vi "LoadCFG.vi"(8 "error in (no error)":errorcluster, 11 "object in":refnum<class "DIO-Configuration.lvclass">) -> (0 "error out":errorcluster, 2 "Success?":bool, 3 "object out":refnum<class "DIO-Configuration.lvclass">)   [LabVIEW 2021, in "DAQmx.lvlib" / "DIO-Configuration.lvclass"]
doc: "Loads Configuration"
uses:
  DIO-Configuration.lvclass
  C:/Users/averna/Documents/LV Gym DEMO/Factory Pattern/Device Channels/Dependencies/Channel.lvlibp/Channel/Configuration_class/Configuration.lvclass
  DIO-Configuration.lvclass/DIO-Configuration.ctl
  Dependencies/Channel.lvlibp/Channel/Configuration_class/properties/ReadConfigurationFile.vi
  <vilib>/Utility/config.llb/Read Key (String).vi
  Dependencies/DIO-Channel.lvlibp/DIO-Configuration_class/DIO-Configuration.lvclass
  <vilib>/Utility/config.llb/NI_LVConfig.lvlib
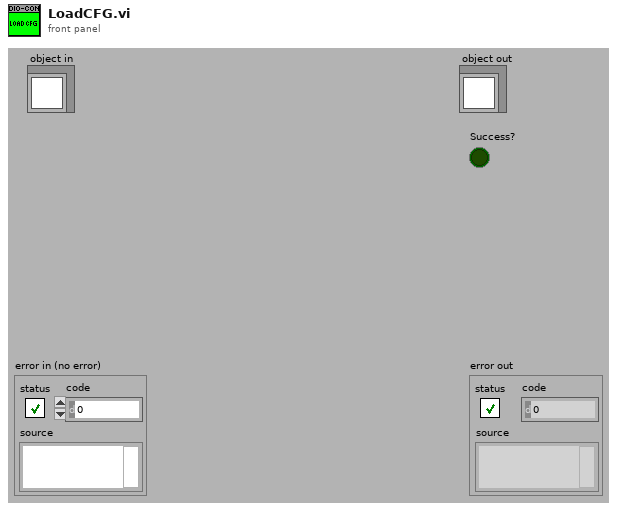
[diagram p1: front panel]
types:
  T1 = typedef "NI_LVConfig.lvlib/Config Data RefNum.ctl" = refnum<k1>
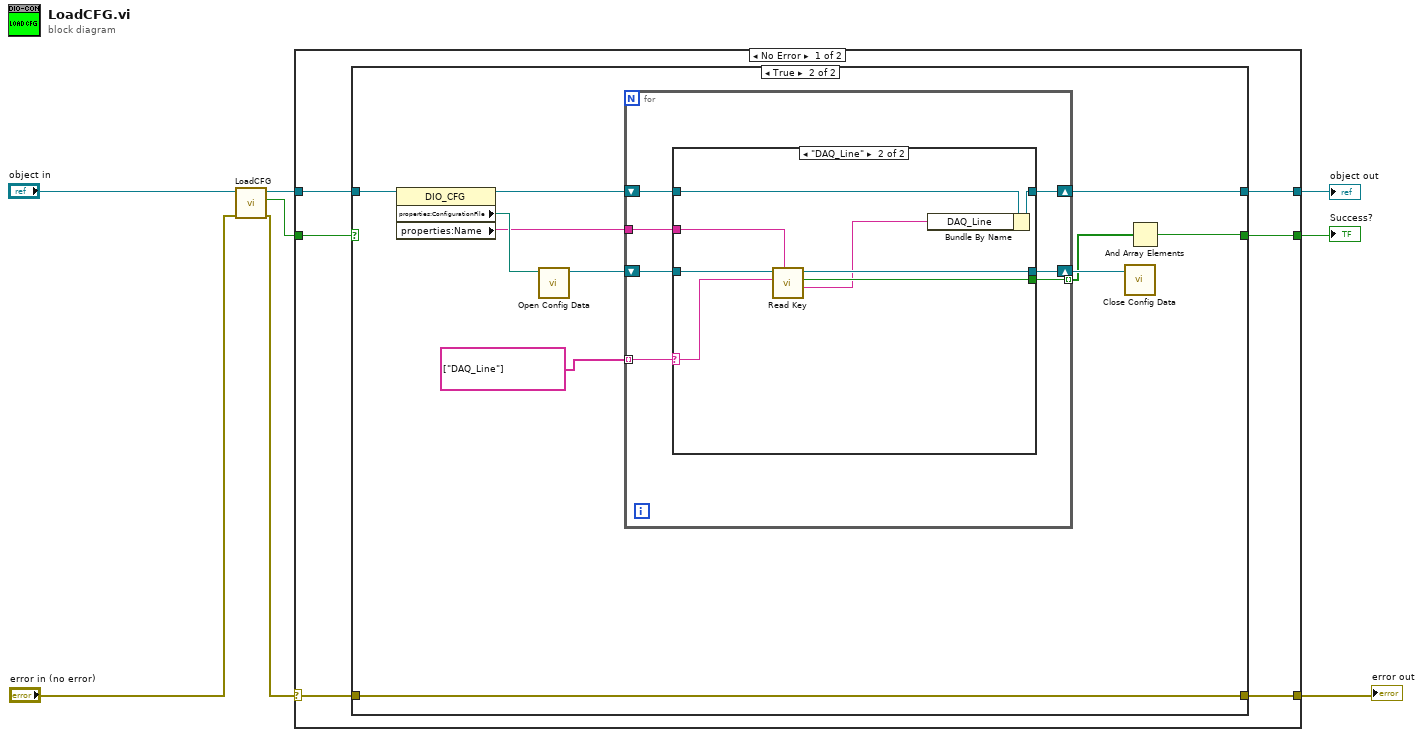
[diagram p0: block diagram]
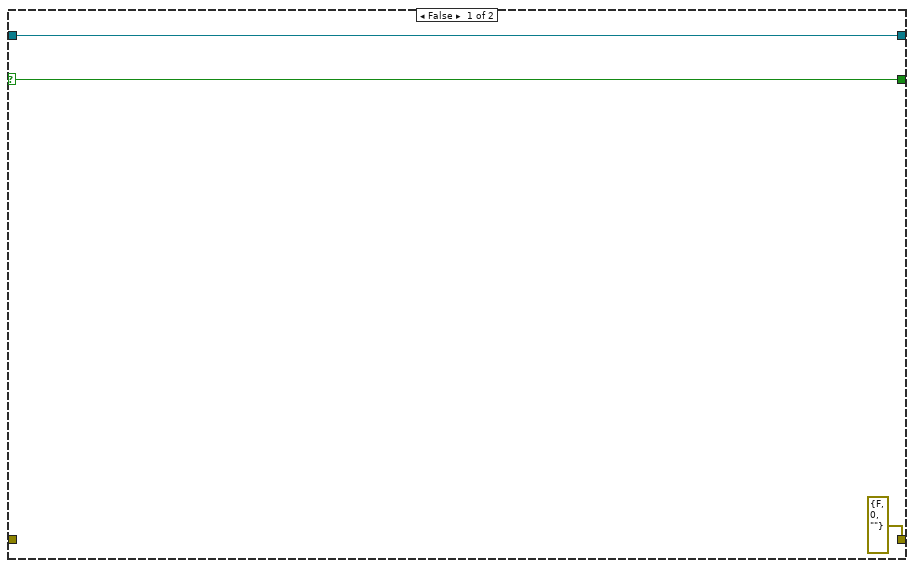
[diagram p2: hidden frame]
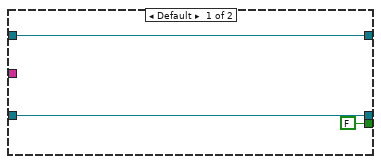
[diagram p3: hidden frame]
diagram:
  n1 = call-parent "LoadCFG.vi"("error in (no error)"="error in (no error)", "object in"="object in") -> ("error out"=w4:errorcluster, "Success?"=w5:bool, "object out"=w6:refnum<class "DIO-Configuration.lvclass">)  [unwired: 7 in]
  n2 = case shown="No Error" w4 {
    selector: w4 -> [w11 w49]
    tunnel: [w12 w49] -> w3
    tunnel: w6 -> [w13 w48]
    tunnel: [w9 w47] -> w1
    tunnel: w5 -> [w10 w47]
    tunnel: [w14 w48] -> w2
    frame No Error {
      n3 = case shown="True" w10 {
        selector: w10 -> [w16 _]
        tunnel: [w17 w24] -> w14
        tunnel: w13 -> [w17 w28]
        tunnel: [errorcluster {"status"=FALSE, "code"=0, "source"=""} ("error IO") w27] -> w12
        tunnel: w11 -> [_ w27]
        tunnel: [w16 w18] -> w9
        frame False {
        }
        frame True {
          n4 = property class="DIO_CFG"(reference=w28) -> (reference out=w23:refnum<class "DIO-Configuration.lvclass">, "properties:ConfigurationFile"=w26:path, "properties:Name"=w20:string)  [unwired: 1 in, 1 out]
          n5 = call <vilib>:"Open Config Data.vi"("configuration file path"=w26) -> ("refnum"=w25:T1)  [unwired: 8 in, 2 out]
          n6 = for {
            shift-right: [w31] -> w24
            shift-left: w23 -> [w30]
            shift-right: [w34] -> w22
            shift-left: w25 -> [w35]
            tunnel: string[] ["DAQ_Line"] -> [w33] mode=indexing
            tunnel: w20 -> [w32]
            tunnel: [w29] -> w19 mode=indexing
            n7 = case shown="\"DAQ_Line\"" w33 {
              selector: w33 -> [_ w44]
              tunnel: w35 -> [w37 w46]
              tunnel: [w37 w45] -> w34
              tunnel: w32 -> [_ w43]
              tunnel: [w38 w40] -> w31
              tunnel: w30 -> [w38 w42]
              tunnel: [FALSE ("found?") w41] -> w29
              frame Default {
              }
              frame "DAQ_Line" {
                n8 = call-poly <vilib>:"Read Key.vi"("section"=w43, "key"=w44, "refnum"=w46) -> ("value"=w39:string, "found?"=w41:bool, "refnum out"=w45:T1)  [unwired: 5 in, 1 out]
                n9 = Bundle By Name(cluster=w42, "DAQ_Line"=w39) -> (w40:refnum<class "DIO-Configuration.lvclass">)
              }
            }
          }
          n10 = call <vilib>:"Close Config Data.vi"("refnum"=w22) -> ()  [unwired: 9 in, 2 out]
          n11 = And Array Elements(Boolean array=w19) -> (logical AND=w18:bool)
        }
      }
    }
    frame Error {
    }
  }
  "error out" <- w3
  "object out" <- w2
  "Success?" <- w1
